vi "MongoDB.GetCollectionNames.vi"(8 "error in (no error)":errorcluster, 11 "MongoDB.Database in":refnum<class "MongoDB.Database.lvclass">) -> (0 "error out":errorcluster, 2 "CollectionNames":string[](array[string]), 3 "MongoDB.Database out":refnum<class "MongoDB.Database.lvclass">)   [LabVIEW 2014, in "MongoDB.Database.lvclass"]
uses:
  MongoDB.Database.lvclass
  MongoDB.Database.lvclass/MongoDB.Database.ctl
  C:/Users/Richard/Documents/GitHub/mongo-labview-driver/CSharp/bin/MongoDB.Driver.Legacy.dll
  CSharp/bin/MongoDB.Driver.Legacy.dll
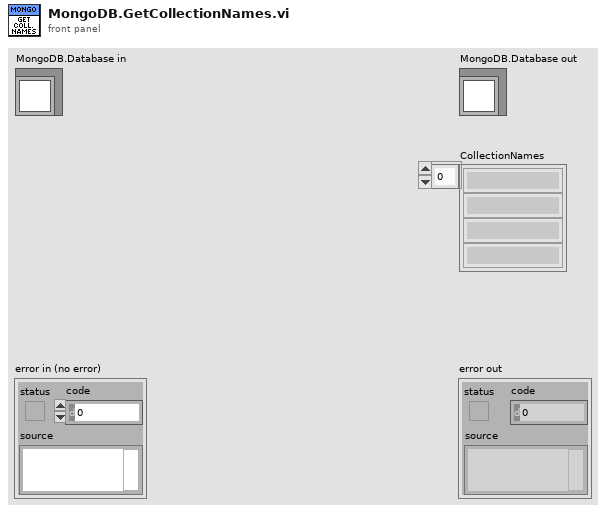
[diagram p1: front panel]
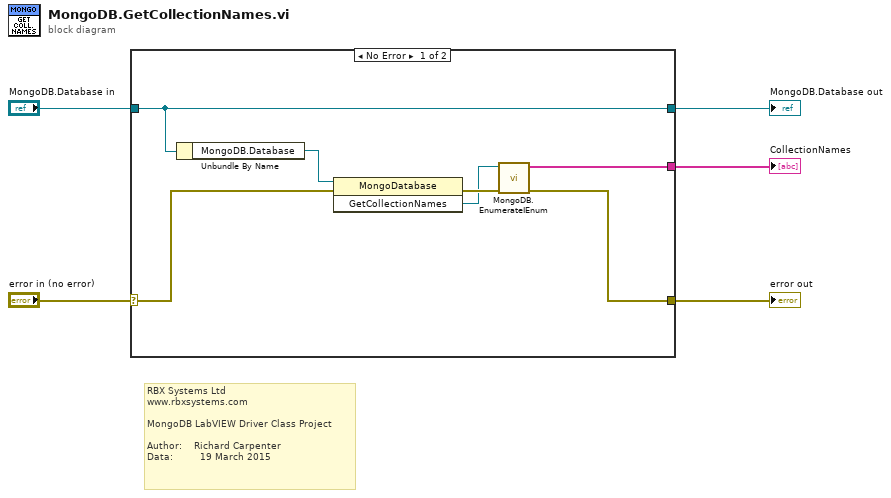
[diagram p0: block diagram]
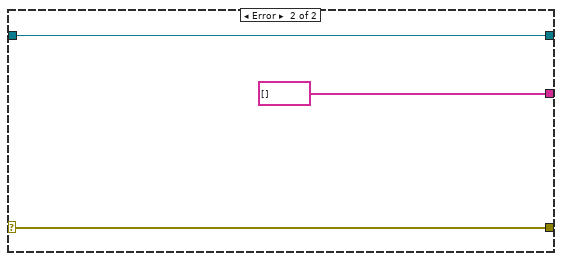
[diagram p2: hidden frame]
diagram:
  # "RBX Systems Ltd\nwww.rbxsystems.com\n\nMongoDB LabVIEW Driver Class Project\n\nAuthor:    Richard Carpenter\nData:         19 March 2015"
  n1 = case shown="No Error" "error in (no error)" {
    selector: "error in (no error)" -> [w12 w15]
    tunnel: [w7 w15] -> w4
    tunnel: [w11 w14] -> w2
    tunnel: "MongoDB.Database in" -> [w11 w14]
    tunnel: [w8 string[] []] -> w1
    frame No Error {
      n2 = Unbundle By Name(w11) -> ("MongoDB.Database"=w10:refnum<k24>)
      n3 = invoke class="MongoDatabase" method="GetCollectionNames"(reference=w10, error in=w12) -> (error out=w9:errorcluster, "GetCollectionNames"=w6:refnum<k24>)  [unwired: 1 in, 1 out]
      n4 = call "MongoDB.EnumerateIEnum.vi"("error in (no error)"=w9, ".NET Refnum in"=w6) -> ("error out"=w7:errorcluster, "Array"=w8:string[])  [unwired: 8 in]
    }
    frame Error {
    }
  }
  "error out" <- w4
  "MongoDB.Database out" <- w2
  "CollectionNames" <- w1
